vi "Stop Condition - Saturation B-Value (SubVI).vi"(6 "Enum":enum16{"Saturation", "B-Check"}(ring), 8 "error in (no error)":errorcluster, 10 "Time":dbl, 11 "Cluster in":T1 {"M Event" items=["Stop", "Running", "PID", "Up Limit", "Down Limit", "Load Limit"]; "Test Type" items=["Please Select"=0, "Triaxial Shear"=1, "Triaxial UU"=2, "Shearbox"=3, "Permeability"=4, "Consolidation (Stepped Loading)/Swelling"=5, "UCT"=8, "Isotropic Consolidation"=9, "Swelling Pressure"=10, "B-Check"=11, "Saturation (Step Increment)"=12, "Saturation (Ramp)"=13]; "Data"."Test Type" items=["Please Select"=0, "Triaxial Shear"=1, "Triaxial UU"=2, "Shearbox"=3, "Permeability"=4, "Consolidation (Stepped Loading)/Swelling"=5, "UCT"=8, "Isotropic Consolidation"=9, "Swelling Pressure"=10, "B-Check"=11, "Saturation (Step Increment)"=12, "Saturation (Ramp)"=13]}) -> (0 "error IO":errorcluster, 3 "Cluster in 2":T1 {"M Event" items=["Stop", "Running", "PID", "Up Limit", "Down Limit", "Load Limit"]; "Test Type" items=["Please Select"=0, "Triaxial Shear"=1, "Triaxial UU"=2, "Shearbox"=3, "Permeability"=4, "Consolidation (Stepped Loading)/Swelling"=5, "UCT"=8, "Isotropic Consolidation"=9, "Swelling Pressure"=10, "B-Check"=11, "Saturation (Step Increment)"=12, "Saturation (Ramp)"=13]; "Data"."Test Type" items=["Please Select"=0, "Triaxial Shear"=1, "Triaxial UU"=2, "Shearbox"=3, "Permeability"=4, "Consolidation (Stepped Loading)/Swelling"=5, "UCT"=8, "Isotropic Consolidation"=9, "Swelling Pressure"=10, "B-Check"=11, "Saturation (Step Increment)"=12, "Saturation (Ramp)"=13]}, 4 "Log?":bool)   [LabVIEW 2019]
uses:
  Controls/RunTest - Data Structure.ctl
  Controls/Test Panel - Data Structure.ctl
  Controls/Station - Test Type.ctl
  <vilib>/Utility/miscctls.llb/LVRowAndColumnTypeDef.ctl
  Controls/RunTest - Calculate Data.ctl
  <vilib>/httpClient/ClientHandle.ctl
  Controls/RunTest - Start Condition.ctl
  Controls/RunTest - Stop Condition.ctl
  Controls/UDP - Event.ctl
  Controls/eFGV States.ctl
  <vilib>/httpClient/LabVIEWHTTPClient.lvlib
panel:
  in  "Test Run Time":dbl
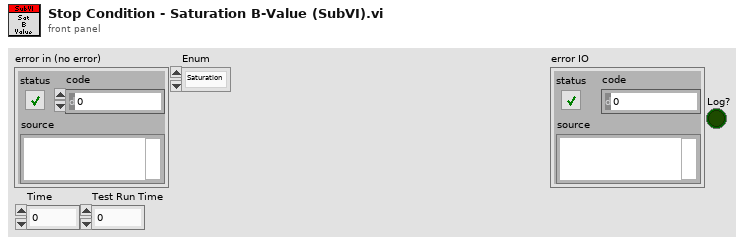
[diagram p1: front panel]
types:
  T1 = typedef "RunTest - Data Structure.ctl" = cluster{"Test Plan":string[], "PlanRow":i32, "Device Name":string[], "Timeout":i32, "Start?":bool, "Pause?":bool, "IP Address":string[], "LogRow":i32, "Logtype":u16, "Log Elapse":sgl, "Data":T2, "Stop log?":bool, "tdms":refnum<k34>, "Sensor Data":sgl[], "Start time":timestamp, "Prev Log Elapse":u32, "Plot":u16, "X-Axis":u16[], "Y-Axis":u16[], "XY":cluster{"X":dbl, "Y":dbl}[][], "End Stage?":bool, "1run":bool, "Condition":u16[], "Start Con":bool, "Log Con":bool, "Stop Con":bool, "Start Elapse":dbl, "Start Load":dbl, "Motor":i32, "StartRow":i32, "number log":i32, "Dir":bool, "Start time test":timestamp, "Auto":bool, "Check return?":bool, "Inv":cluster{"M":i32[], "Bool":bool[]}, "tdms temp":refnum<k34>, "Zero?":bool, "Plot Timer":dbl, "1st Run":bool, "TDMS Path":path, "MaxLoad":dbl, "Log Timer":sgl[], "Test Type":T3, "Log Sensor":string[], "Save?":bool, "1st Log":bool, "Y-Axis 2":u16[], "On Y-Axis 2":bool, "Decimal":u8[], "Init":cluster{"PWP TS":sgl, "Load TS":sgl, "Volume TS":sgl, "Disp TS":sgl, "CP":sgl, "Vol In":sgl, "Vol Out":sgl, "Load UCT":sgl, "Disp UCT":sgl, "PWP Sat":sgl, "CP Sat":sgl, "Volume IsoCons":sgl, "PWP IsoCons":sgl, "PWP TUU":sgl, "Load TUU":sgl, "Volume TUU":sgl, "Disp TUU":sgl, "Load Cons":sgl, "Disp Cons":sgl, "Volume Sat":sgl, "Vertical Load SB":sgl, "Vertical Disp SB":sgl, "H Disp SB":sgl, "H Load SB":sgl, "PWP BC":sgl, "CP BC":sgl, "PWP Sat Step":sgl, "CP Sat Step":sgl, "Volume Sat Step":sgl, "PWP Sat Ramp":sgl, "CP Sat Ramp":sgl, "Volume Sat Ramp":sgl}, "Calc":T5, "Device Index":i32[], "Channel Index":i32[], "http ref":T6, "fileid":string, "Step Cons":cluster{"V Stress":sgl, "H Settlement":sgl}, "RunTest":bool, "Graph Last":i32, "Init?":bool, "Datalog":bool[], "Start":T7, "Stop":T8, "Running?":bool, "StartTime":dbl, "Log Prev Time":dbl, "KeyName":string[], "Test RunTime":dbl, "Log Prev Axial":dbl, "M Event":T9[], "Last Log":bool, "popup":bool, "PreStart UU":bool, "PreStart Sat":bool, "PreStart BC":bool, "PreStart Sat Step":bool, "PreStart Sat Ramp":bool, "Prev Sat IP":string, "IP Device ID":string[]}
  T2 = typedef "Test Panel - Data Structure.ctl" = cluster{"Station":string, "Sample ID":string, "Job No":string, "Job Description":string, "Filename":string, "Test Type":T3, "Speciment No":string, "Depth":string, "Height":string, "Diameter/Length":string, "Weight":string, "Test Parameter":string, "Station[]":string[], "Edit Pos":T4, "Edit Pos Prev":T4, "Area":string, "Path":string, "sample_id":string}
  T3 = typedef "Station - Test Type.ctl" = u16
  T4 = typedef "LVRowAndColumnTypeDef.ctl" = cluster{"Row":i32, "Column":i32}
  T5 = typedef "RunTest - Calculate Data.ctl" = cluster{"TS":cluster{"Change PWP":sgl, "Change Vol":sgl, "Axial Load":sgl, "CiL":sgl, "Deviator":sgl, "Axial Strain":sgl, "MaxDeviator":sgl, "SS":sgl, "CAS":sgl}, "TUU":cluster{"Change PWP":sgl, "Axial Load":sgl, "CiL":sgl, "Deviator":sgl, "Axial Strain":sgl, "MaxDeviator":sgl}, "Sat":cluster{"B Value":sgl, "PWP Diss":sgl, "CPP":sgl, "CV":sgl}, "Per":cluster{"Change Vol In":sgl, "Change Vol Out":sgl, "Mean Vol":sgl, "Gradient Pressure":sgl, "Outlet Flow":sgl, "Inlet Flow":sgl, "I X1":sgl, "I X2":sgl, "I Y1":sgl, "I Y2":sgl, "O X1":sgl, "O X2":sgl, "O Y1":sgl, "O Y2":sgl}, "Step Cons":cluster{"V Stress":sgl, "H Settlement":sgl, "Total H Settle":sgl, "Prev Total H":sgl}, "UCT":cluster{"ALC":sgl, "H Change":sgl, "Deviator":sgl, "Axial Strain":sgl, "V Stress":sgl, "MaxDeviator":sgl}, "ISO Cons":cluster{"CPP":sgl, "PWP Diss":sgl, "CV":sgl, "VS":sgl}, "SB":cluster{"Speci LenC":sgl, "Shear Strain":sgl, "H LC":sgl, "Normal Stress":sgl, "Shear Stress":sgl, "MaxShear":sgl}, "BC":cluster{"B Value":sgl, "PWP Diss":sgl, "CPP":sgl, "CV":sgl}, "Sat Step":cluster{"B Value":sgl, "PWP Diss":sgl, "CPP":sgl, "CV":sgl}, "Sat Ramp":cluster{"B Value":sgl, "PWP Diss":sgl, "CPP":sgl, "CV":sgl}, "Prev Log":string[]}
  T6 = typedef "LabVIEWHTTPClient.lvlib/ClientHandle.ctl" = refnum<k1>
  T7 = typedef "RunTest - Start Condition.ctl" = cluster{"Cons":cluster{"VS":dbl, "Delay":bool, "No Delay":dbl}, "Sat":cluster{"CP":dbl, "BP":dbl, "StartBP":bool, "Target CP":bool, "Target BP":bool}, "Iso":cluster{"Select":dbl, "BP":dbl, "IC2":dbl, "IC3":dbl, "IC4":dbl, ". IC6":bool, "IC6":dbl, "IC6-2":dbl, "Time Cond":dbl, "Last PWP":dbl, "Target CP":bool, "Target BP":bool, "NewCP":dbl, "NewBP":dbl, "Noti CP":bool, "Noti BP":bool, "Noti PWP":bool, "PrevSatBP":dbl}, "TS":cluster{"SS":dbl, "Engage":bool, "ES":dbl, "LC":dbl, "PreStart":bool, "Trig SS":bool, "Drain":dbl, "Select":u16, "Max SS .":bool, "MaxSS":dbl}, "TUU":cluster{"SS":dbl, "Engage":bool, "ES":dbl, "LC":dbl, "PreStart":bool, "Trig SS":bool, "CP":dbl, "Delay Value":dbl, "Delay":bool, "CP PID":bool}, "UCT":cluster{"SS":dbl, "Engage":bool, "ES":dbl, "LC":dbl, "PreStart":bool, "Trig SS":bool}, "Enable?":bool, "SB":cluster{"SS":dbl, "Engage":bool, "ES":dbl, "LC":dbl, "PreStart":bool, "Trig SS":bool, "VS":dbl, "Delay Value":dbl, "Delay":bool, "VS PID":bool}, "Perm":cluster{"DP":dbl}, "BC":cluster{"CP":dbl, "Target CP":bool, "Target BP":bool, "CP Inc":dbl, "CP .Init":bool, "CP Init":dbl, "1st BC":bool}, "Sat (Step)":cluster{"Select":dbl, "CP":dbl, "BP":dbl, "EP":dbl, "StartCP":bool, "Target CP":bool, "Target BP":bool}, "Sat (Ramp)":cluster{"Select":dbl, "CP":dbl, "BP":dbl, "EP":dbl, "StartCP":bool, "Target CP":bool, "Target BP":bool, "Time Rate":u32}}
  T8 = typedef "RunTest - Stop Condition.ctl" = cluster{"Cons":cluster{"Select":i32, "Disp":dbl, "Time":dbl, "Time2":dbl, "Disp 2":dbl, "Time Cond":dbl, "Last Disp":dbl, "Swell":bool, "T50,90,100":cluster{"t50_x_min":dbl, "t50_y_value":dbl, "t90_x_min":dbl, "t90_y_value":dbl, "t100_x_min":dbl, "t100_y_value":dbl, "target_column":string, "test_type":string, "error":string}}, "Sat":cluster{"Select":i32, "PP":dbl, "Time":dbl, "VC":dbl, "Time2":dbl, "Time Cond":dbl, "Last PP":dbl, ".B":bool, "B":dbl, "Last Vc":dbl, "Time Cond 2":dbl, "Time3":dbl, "Time Cond 3":dbl, "B Achieve":bool, "PP Achieve":bool, "VC Achieve":bool, "Max Achieve":bool, "CP Check":dbl, "Skip Next":bool, "B Achieve Stage":u32, ".CP Check":bool}, "Iso":cluster{"PP":dbl, "Time":dbl, "VC":dbl, "Time2":dbl, "Time Cond":dbl, "Last Vc":dbl, ".PP":bool, "Time Cond 2":dbl, "Select":i32, "BS":cluster{"t50_x_min":dbl, "t50_y_value":dbl, "t90_x_min":dbl, "t90_y_value":dbl, "t100_x_min":dbl, "t100_y_value":dbl, "target_column":string, "test_type":string, "error":string}, "Final VC":dbl, "ASTM":cluster{"t50_x_min":dbl, "t50_y_value":dbl, "t90_x_min":dbl, "t90_y_value":dbl, "t100_x_min":dbl, "t100_y_value":dbl, "target_column":string, "test_type":string, "error":string}, "ASTM Log":cluster{"t50_x_min":dbl, "t50_y_value":dbl, "t90_x_min":dbl, "t90_y_value":dbl, "t100_x_min":dbl, "t100_y_value":dbl, "target_column":string, "test_type":string, "error":string}, "PP Achieve":bool, "VC Achieve":bool}, "TS":cluster{"Axial":dbl, ".MaxDev":bool, "MaxDev Value":dbl, "Return":bool, "Reset":bool, "Prev Time":dbl, "PostStop Run":bool, "CP Stop":bool, "BP Stop":bool, "PostStop Trig":bool, "Reset Value":dbl, "BPTrig":bool, "CPTrig":bool, "VLCTrig":bool, "CAxial":dbl, "Select":i32}, "TUU":cluster{"Axial":dbl, ".MaxDev":bool, "MaxDev Value":dbl, "Return":bool, "Reset":bool, "Prev Time":dbl, "PostStop Run":bool, "CP Stop":bool, "BP Stop":bool, "PostStop Trig":bool, "Reset Value":dbl, "BPTrig":bool, "CPTrig":bool, "VLCTrig":bool}, "UCT":cluster{"Axial":dbl, ".MaxDev":bool, "MaxDev Value":dbl, "Return":bool, "Reset":bool, "Prev Time":dbl, "PostStop Run":bool, "CP Stop":bool, "BP Stop":bool, "PostStop Trig":bool}, "Enable?":bool, "SB":cluster{"Shear":dbl, ".MaxShear":bool, "MaxShear Value":dbl, "Return":bool, "Reset":bool, "Prev Time":dbl, "PostStop Run":bool, "CP Stop":bool, "BP Stop":bool, "PostStop Trig":bool, "Reset Value":dbl, "BPTrig":bool, "CPTrig":bool, "VLCTrig":bool}, "Perm":cluster{"Max Time":bool, "Reset":bool, "PostStop Run":bool, "Ratio":bool, "Reset Value":dbl, "Time":dbl, "RatioTime":dbl, "RatioMore":dbl, "RatioLess":dbl, "Time Cond":dbl, "Time Cond 2":dbl, "Prev IF":dbl, "Prev OF":dbl, "PostStop Trig":bool, "BP Trig":bool, "DP Stop":bool, "BP Stop":bool, "CP Stop":bool, "CP Trig":bool}, "SP":cluster{".Max Time":bool, ".Time":bool, "Time":dbl, "MaxTime":dbl, "Time Cond":dbl, "Max Time Cond":dbl, "Stress":dbl}, "BC":cluster{"Select":i32, "PP":dbl, "Time":dbl, "Time Cond":dbl, "Last PP":dbl, ".B":bool, "B":dbl, "Time 2":dbl, "Time Cond 2":dbl, "B Achieve":bool, "PP Achieve":bool, "Max Achieve":bool, "CP Check":dbl, "Skip Next":bool, "B Achieve Stage":u32, ".CP Check":bool}, "Sat (Step)":cluster{"Select":i32, "PP":dbl, "Time":dbl, "VC":dbl, "Time2":dbl, "Time Cond":dbl, "Last PP":dbl, ".B":bool, "B":dbl, "Last Vc":dbl, "Time Cond 2":dbl, "Time3":dbl, "Time Cond 3":dbl, "B Achieve":bool, "PP Achieve":bool, "VC Achieve":bool, "Max Achieve":bool, "CP Check":dbl, "Skip Next":bool, "B Achieve Stage":u32}, "Sat (Ramp)":cluster{"Select":i32, "PP":dbl, "Time":dbl, "VC":dbl, "Time2":dbl, "Time Cond":dbl, "Last PP":dbl, ".B":bool, "B":dbl, "Last Vc":dbl, "Time Cond 2":dbl, "Time3":dbl, "Time Cond 3":dbl, "B Achieve":bool, "PP Achieve":bool, "VC Achieve":bool, "Max Achieve":bool, "CP Check":dbl, "Skip Next":bool, "B Achieve Stage":u32}}
  T9 = typedef "UDP - Event.ctl" = u16
  T10 = typedef "eFGV States.ctl" = enum16{"Init", "Read", "Write", "Exit"}
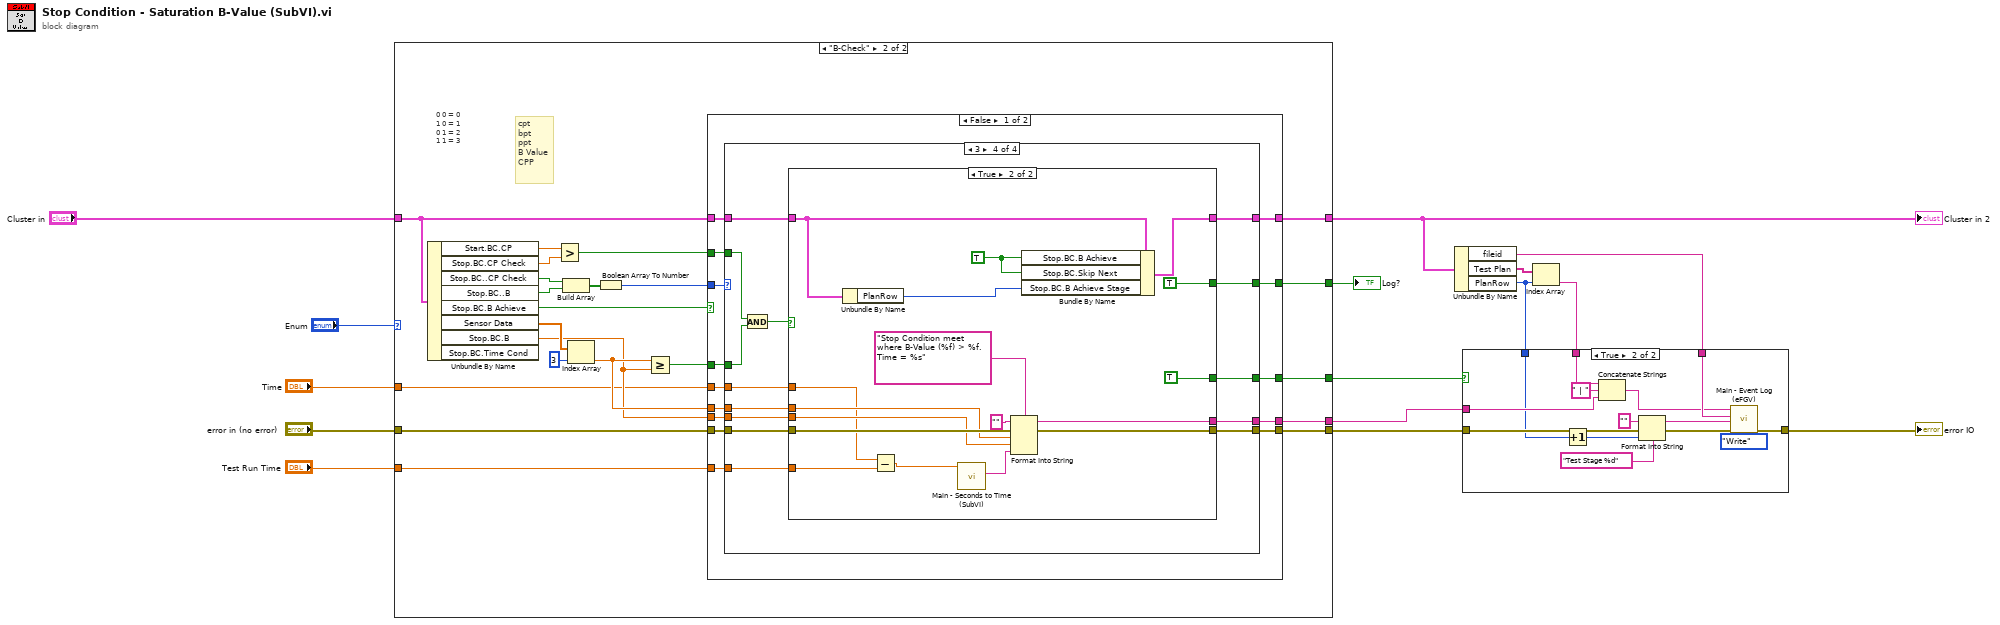
[diagram p0: block diagram]
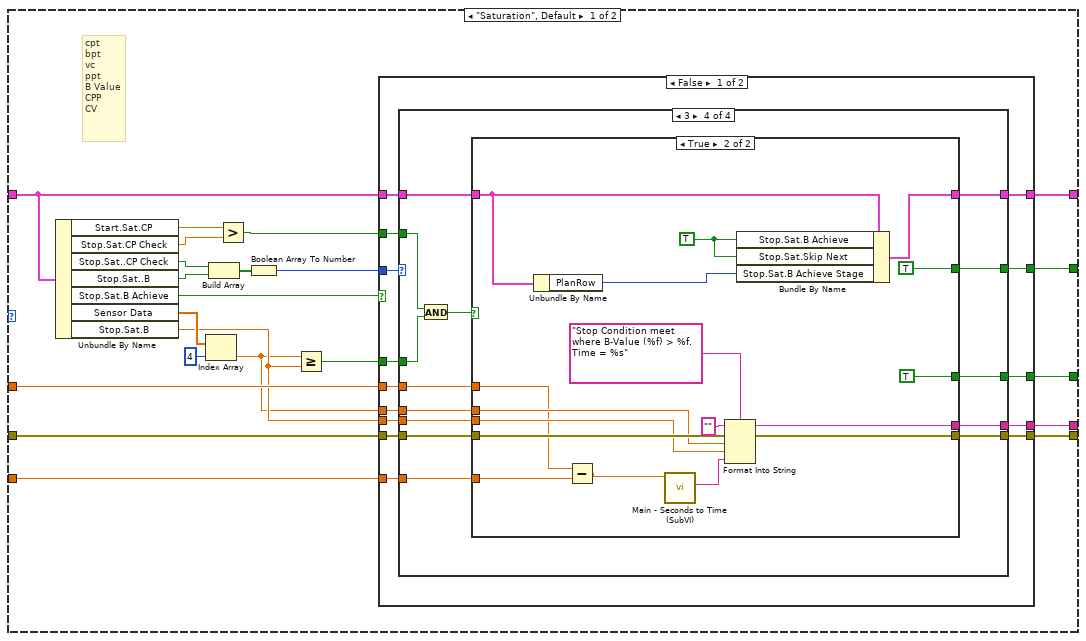
[diagram p2: hidden frame]
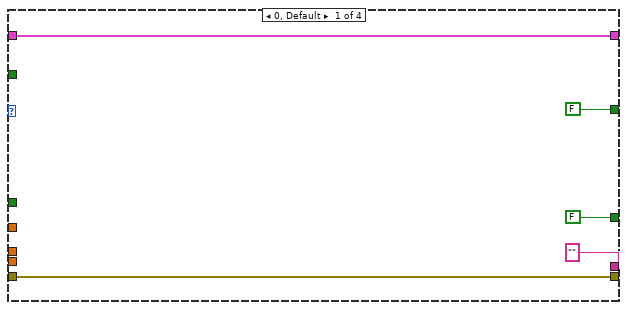
[diagram p3: hidden frame]
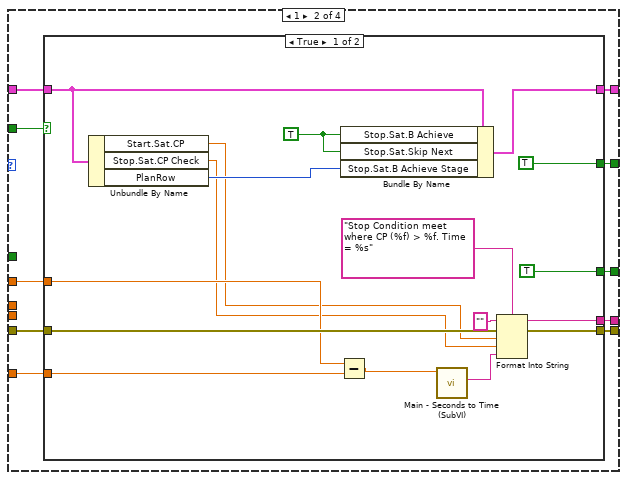
[diagram p4: hidden frame]
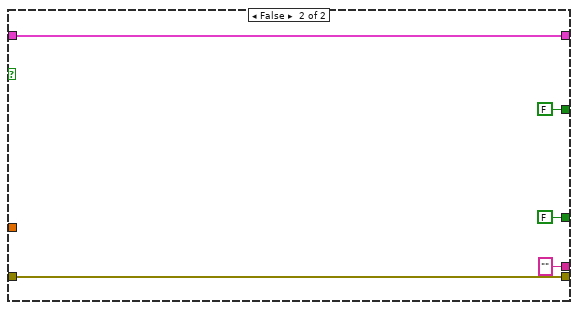
[diagram p5: hidden frame]
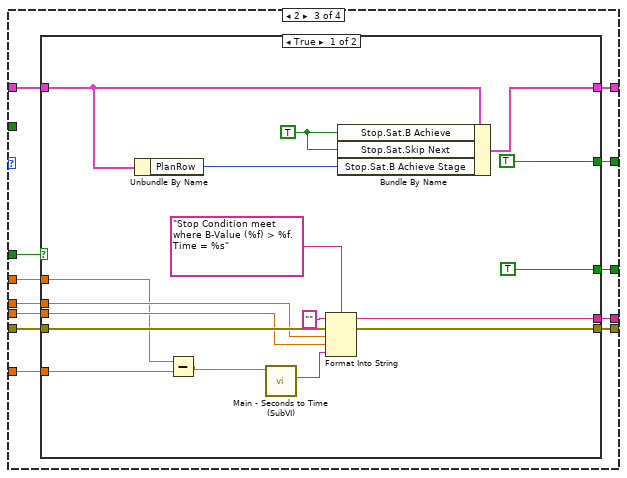
[diagram p6: hidden frame]
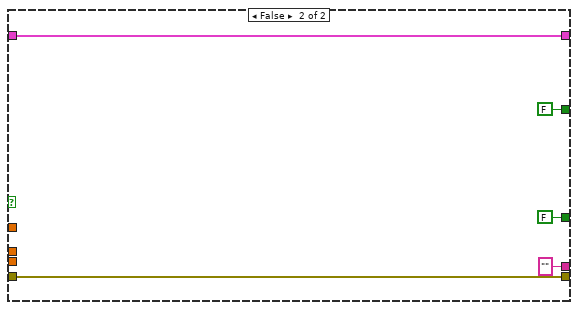
[diagram p7: hidden frame]
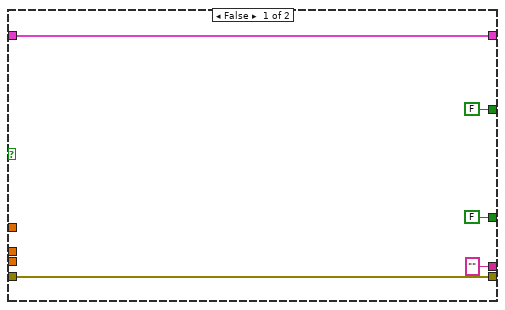
[diagram p8: hidden frame]
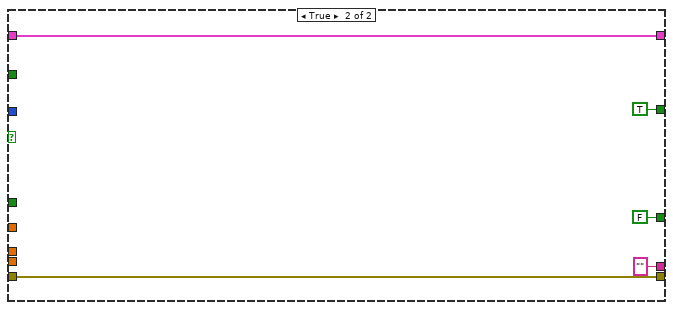
[diagram p9: hidden frame]
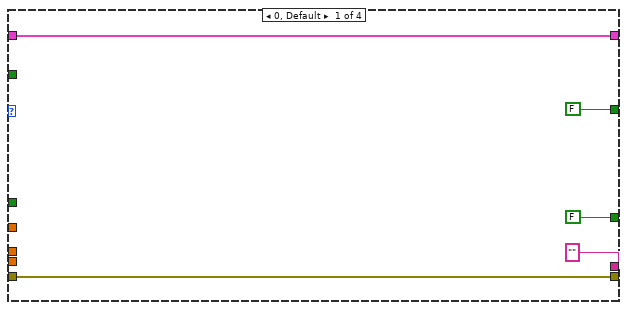
[diagram p10: hidden frame]
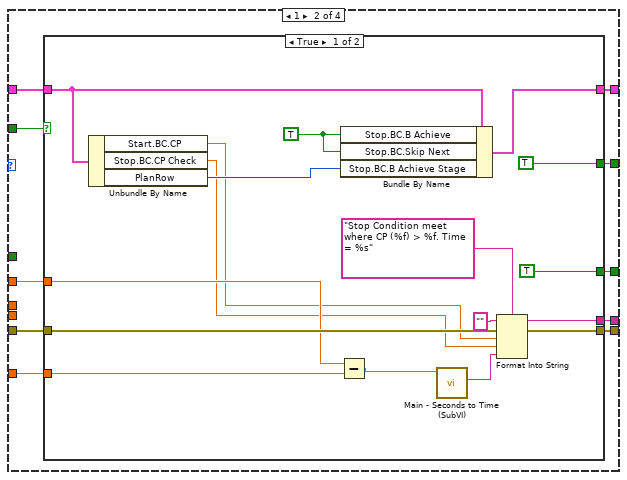
[diagram p11: hidden frame]
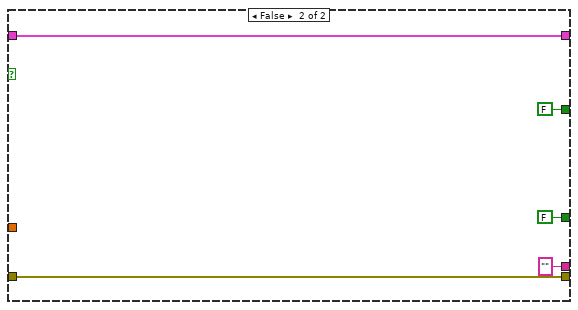
[diagram p12: hidden frame]
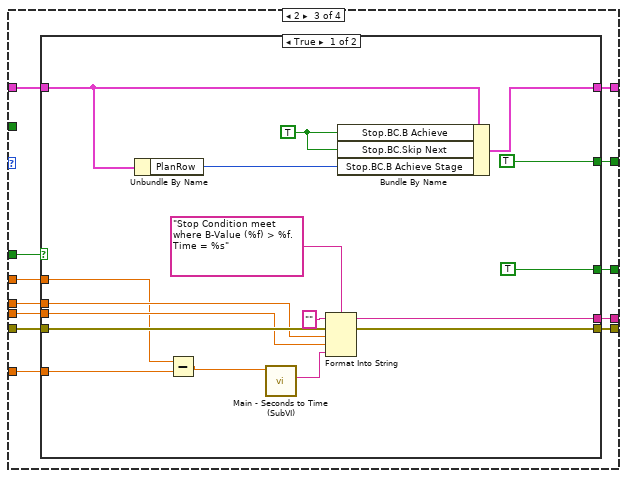
[diagram p13: hidden frame]
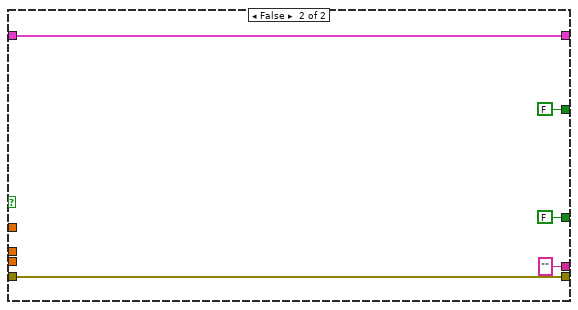
[diagram p14: hidden frame]
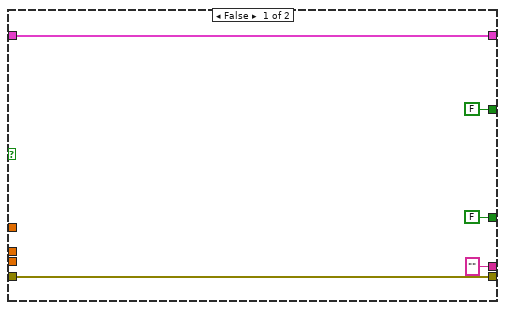
[diagram p15: hidden frame]
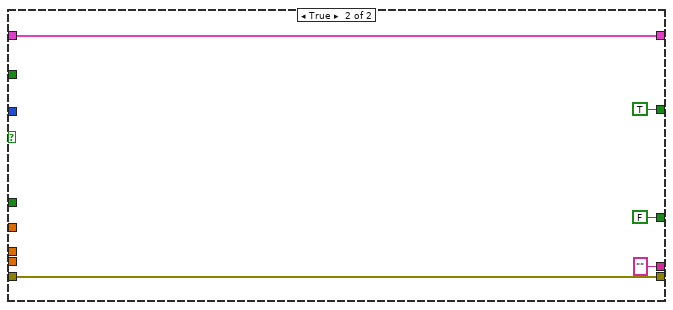
[diagram p16: hidden frame]
diagram:
  n1 = case shown="\"B-Check\"" "Enum" {
    tunnel: "Cluster in" -> [w30 w176]
    tunnel: "error in (no error)" -> [w35 w172]
    tunnel: "Time" -> [w33 w164]
    tunnel: [w21 w175] -> w12
    tunnel: [w18 w173] -> w7
    tunnel: [w20 w174] -> w6
    tunnel: [w22 w177] -> w5
    tunnel: [w19 w171] -> w3
    tunnel: "Test Run Time" -> [w34 w169]
    frame "Saturation", Default {
      # "cpt\nbpt\nvc\nppt\nB Value\nCPP\nCV"
      n2 = Unbundle By Name(w30) -> ("Start.Sat.CP"=w32:dbl, "Stop.Sat.CP Check"=w31:dbl, "Stop.Sat..CP Check"=w25:bool, "Stop.Sat..B"=w24:bool, "Stop.Sat.B Achieve"=w27:bool, "Sensor Data"=w37:sgl[], "Stop.Sat.B"=w17:dbl)
      n3 = Index Array(array=w37, index=4) -> (element=w16:sgl)
      n4 = Build Array(w25, w24) -> (w26:bool[])
      n5 = Greater?(x=w32, y=w31) -> (0:w29:bool)
      n6 = Boolean Array To Number(Boolean array=w26) -> (number=w23:u32)
      n7 = Greater Or Equal?(x=w16, y=w17) -> (x >= y?=w28:bool)
      n8 = case shown="False" w27 {
        tunnel: w23 -> [w51 _]
        tunnel: [w50 w163] -> w22
        tunnel: w30 -> [w49 w163]
        tunnel: [w48 TRUE] -> w21
        tunnel: [w47 FALSE] -> w20
        tunnel: [w46 w160] -> w18
        tunnel: w35 -> [w45 w160]
        tunnel: [w44 ""] -> w19
        tunnel: w29 -> [w43 _]
        tunnel: w33 -> [w42 _]
        tunnel: w34 -> [w41 _]
        tunnel: w28 -> [w40 _]
        tunnel: w16 -> [w39 _]
        tunnel: w17 -> [w38 _]
        frame False {
          n9 = case shown="3" w51 {
            tunnel: [w56 w65 w99 w129] -> w50
            tunnel: w49 -> [w56 w66 w100 w130]
            tunnel: [FALSE w64 w97 w128] -> w48
            tunnel: [FALSE w63 w96 w127] -> w47
            tunnel: [w53 w61 w94 w135] -> w46
            tunnel: w45 -> [w53 w60 w93 w136]
            tunnel: ["" w62 w95 w126] -> w44
            tunnel: w43 -> [_ w59 _ w125]
            tunnel: w42 -> [_ w58 w92 w131]
            tunnel: w41 -> [_ w57 w91 w132]
            tunnel: w40 -> [_ _ w98 w124]
            tunnel: w39 -> [_ _ w90 w134]
            tunnel: w38 -> [_ _ w89 w133]
            frame 0, Default {
            }
            frame 1 {
              n10 = case shown="True" w59 {
                tunnel: [w81 w85] -> w61
                tunnel: w60 -> [w82 w85]
                tunnel: [w83 w88] -> w65
                tunnel: w66 -> [w77 w88]
                tunnel: [w79 ""] -> w62
                tunnel: [TRUE FALSE] -> w63
                tunnel: w58 -> [w76 _]
                tunnel: [TRUE FALSE] -> w64
                tunnel: w57 -> [w75 _]
                frame True {
                  w67 = TRUE ("Stop.Sat.B Achieve")
                  n11 = Unbundle By Name(w77) -> ("Start.Sat.CP"=w73:dbl, "Stop.Sat.CP Check"=w72:dbl, "PlanRow"=w74:i32)
                  n12 = Subtract(x=w76, y=w75) -> (x-y=w68:dbl)
                  n13 = Bundle By Name(cluster=w77, "Stop.Sat.B Achieve"=w67, "Stop.Sat.Skip Next"=w67, "Stop.Sat.B Achieve Stage"=w74) -> (w83:T1)
                  n14 = call "Main - Seconds to Time (SubVI).vi"("Seconds"=w68) -> ("Time string"=w69:string)  [unwired: 9 in, 1 out]
                  n15 = Format Into String(format string="Stop Condition meet where CP (%f) > %f. Time = %s", initial string="", error in=w82, w73, w72, w69) -> (resulting string=w79:string, error out=w81:errorcluster)
                }
                frame False {
                }
              }
            }
            frame 2 {
              n16 = case shown="True" w98 {
                tunnel: [w115 w121] -> w94
                tunnel: w93 -> [w116 w121]
                tunnel: [w117 w122] -> w99
                tunnel: w100 -> [w109 w122]
                tunnel: w89 -> [w114 _]
                tunnel: w90 -> [w113 _]
                tunnel: [w111 ""] -> w95
                tunnel: [TRUE FALSE] -> w96
                tunnel: w92 -> [w108 _]
                tunnel: [TRUE FALSE] -> w97
                tunnel: w91 -> [w107 _]
                frame True {
                  w101 = TRUE ("Stop.Sat.B Achieve")
                  n17 = Unbundle By Name(w109) -> ("PlanRow"=w103:i32)
                  n18 = Subtract(x=w108, y=w107) -> (x-y=w102:dbl)
                  n19 = call "Main - Seconds to Time (SubVI).vi"("Seconds"=w102) -> ("Time string"=w104:string)  [unwired: 9 in, 1 out]
                  n20 = Format Into String(format string="Stop Condition meet where B-Value (%f) > %f. Time = %s", initial string="", error in=w116, w113, w114, w104) -> (resulting string=w111:string, error out=w115:errorcluster)
                  n21 = Bundle By Name(cluster=w109, "Stop.Sat.B Achieve"=w101, "Stop.Sat.Skip Next"=w101, "Stop.Sat.B Achieve Stage"=w103) -> (w117:T1)
                }
                frame False {
                }
              }
            }
            frame 3 {
              n22 = And(x=w125, y=w124) -> (x .and. y?=w123:bool)
              n23 = case shown="True" w123 {
                tunnel: [w141 w158] -> w129
                tunnel: w136 -> [w138 w155]
                tunnel: [w138 w154] -> w135
                tunnel: w133 -> [_ w153]
                tunnel: w134 -> [_ w152]
                tunnel: [FALSE TRUE] -> w127
                tunnel: ["" w149] -> w126
                tunnel: [FALSE TRUE] -> w128
                tunnel: w130 -> [w141 w147]
                tunnel: w131 -> [_ w144]
                tunnel: w132 -> [_ w143]
                frame False {
                }
                frame True {
                  w142 = TRUE ("Stop.Sat.B Achieve")
                  n24 = Unbundle By Name(w147) -> ("PlanRow"=w146:i32)
                  n25 = Subtract(x=w144, y=w143) -> (x-y=w145:dbl)
                  n26 = call "Main - Seconds to Time (SubVI).vi"("Seconds"=w145) -> ("Time string"=w150:string)  [unwired: 9 in, 1 out]
                  n27 = Format Into String(format string="Stop Condition meet where B-Value (%f) > %f. Time = %s", initial string="", error in=w155, w152, w153, w150) -> (resulting string=w149:string, error out=w154:errorcluster)
                  n28 = Bundle By Name(cluster=w147, "Stop.Sat.B Achieve"=w142, "Stop.Sat.Skip Next"=w142, "Stop.Sat.B Achieve Stage"=w146) -> (w158:T1)
                }
              }
            }
          }
        }
        frame True {
        }
      }
    }
    frame "B-Check" {
      # "0 0 = 0\n1 0 = 1\n0 1 = 2\n1 1 = 3"
      # "cpt\nbpt\nppt\nB Value\nCPP"
      n29 = Unbundle By Name(w176) -> ("Start.BC.CP"=w183:dbl, "Stop.BC.CP Check"=w182:dbl, "Stop.BC..CP Check"=w181:bool, "Stop.BC..B"=w180:bool, "Stop.BC.B Achieve"=w165:bool, "Sensor Data"=w185:sgl[], "Stop.BC.B"=w166:dbl)  [unwired: 1 out]
      n30 = Greater?(x=w183, y=w182) -> (0:w170:bool)
      n31 = Build Array(w181, w180) -> (w179:bool[])
      n32 = Index Array(array=w185, index=3) -> (element=w167:sgl)
      n33 = Boolean Array To Number(Boolean array=w179) -> (number=w178:u32)
      n34 = Greater Or Equal?(x=w167, y=w166) -> (x >= y?=w168:bool)
      n35 = case shown="False" w165 {
        tunnel: w178 -> [w199 _]
        tunnel: [w198 w311] -> w177
        tunnel: w176 -> [w197 w311]
        tunnel: [w196 TRUE] -> w175
        tunnel: [w195 FALSE] -> w174
        tunnel: [w194 w308] -> w173
        tunnel: w172 -> [w193 w308]
        tunnel: [w192 ""] -> w171
        tunnel: w170 -> [w191 _]
        tunnel: w164 -> [w190 _]
        tunnel: w169 -> [w189 _]
        tunnel: w168 -> [w188 _]
        tunnel: w167 -> [w187 _]
        tunnel: w166 -> [w186 _]
        frame False {
          n36 = case shown="3" w199 {
            tunnel: [w204 w213 w247 w277] -> w198
            tunnel: w197 -> [w204 w214 w248 w278]
            tunnel: [FALSE w212 w245 w276] -> w196
            tunnel: [FALSE w211 w244 w275] -> w195
            tunnel: [w201 w209 w242 w283] -> w194
            tunnel: w193 -> [w201 w208 w241 w284]
            tunnel: ["" w210 w243 w274] -> w192
            tunnel: w191 -> [_ w207 _ w273]
            tunnel: w190 -> [_ w206 w240 w279]
            tunnel: w189 -> [_ w205 w239 w280]
            tunnel: w188 -> [_ _ w246 w272]
            tunnel: w187 -> [_ _ w238 w282]
            tunnel: w186 -> [_ _ w237 w281]
            frame 0, Default {
            }
            frame 1 {
              n37 = case shown="True" w207 {
                tunnel: [w229 w233] -> w209
                tunnel: w208 -> [w230 w233]
                tunnel: [w231 w236] -> w213
                tunnel: w214 -> [w225 w236]
                tunnel: [w227 ""] -> w210
                tunnel: [TRUE FALSE] -> w211
                tunnel: w206 -> [w224 _]
                tunnel: [TRUE FALSE] -> w212
                tunnel: w205 -> [w223 _]
                frame True {
                  w215 = TRUE ("Stop.Sat.B Achieve")
                  n38 = Unbundle By Name(w225) -> ("Start.BC.CP"=w221:dbl, "Stop.BC.CP Check"=w220:dbl, "PlanRow"=w222:i32)
                  n39 = Subtract(x=w224, y=w223) -> (x-y=w216:dbl)
                  n40 = Bundle By Name(cluster=w225, "Stop.BC.B Achieve"=w215, "Stop.BC.Skip Next"=w215, "Stop.BC.B Achieve Stage"=w222) -> (w231:T1)
                  n41 = call "Main - Seconds to Time (SubVI).vi"("Seconds"=w216) -> ("Time string"=w217:string)  [unwired: 9 in, 1 out]
                  n42 = Format Into String(format string="Stop Condition meet where CP (%f) > %f. Time = %s", initial string="", error in=w230, w221, w220, w217) -> (resulting string=w227:string, error out=w229:errorcluster)
                }
                frame False {
                }
              }
            }
            frame 2 {
              n43 = case shown="True" w246 {
                tunnel: [w263 w269] -> w242
                tunnel: w241 -> [w264 w269]
                tunnel: [w265 w270] -> w247
                tunnel: w248 -> [w257 w270]
                tunnel: w237 -> [w262 _]
                tunnel: w238 -> [w261 _]
                tunnel: [w259 ""] -> w243
                tunnel: [TRUE FALSE] -> w244
                tunnel: w240 -> [w256 _]
                tunnel: [TRUE FALSE] -> w245
                tunnel: w239 -> [w255 _]
                frame True {
                  w249 = TRUE ("Stop.Sat.B Achieve")
                  n44 = Unbundle By Name(w257) -> ("PlanRow"=w251:i32)
                  n45 = Subtract(x=w256, y=w255) -> (x-y=w250:dbl)
                  n46 = call "Main - Seconds to Time (SubVI).vi"("Seconds"=w250) -> ("Time string"=w252:string)  [unwired: 9 in, 1 out]
                  n47 = Format Into String(format string="Stop Condition meet where B-Value (%f) > %f. Time = %s", initial string="", error in=w264, w261, w262, w252) -> (resulting string=w259:string, error out=w263:errorcluster)
                  n48 = Bundle By Name(cluster=w257, "Stop.BC.B Achieve"=w249, "Stop.BC.Skip Next"=w249, "Stop.BC.B Achieve Stage"=w251) -> (w265:T1)
                }
                frame False {
                }
              }
            }
            frame 3 {
              n49 = And(x=w273, y=w272) -> (x .and. y?=w271:bool)
              n50 = case shown="True" w271 {
                tunnel: [w289 w306] -> w277
                tunnel: w284 -> [w286 w303]
                tunnel: [w286 w302] -> w283
                tunnel: w281 -> [_ w301]
                tunnel: w282 -> [_ w300]
                tunnel: [FALSE TRUE] -> w275
                tunnel: ["" w297] -> w274
                tunnel: [FALSE TRUE] -> w276
                tunnel: w278 -> [w289 w295]
                tunnel: w279 -> [_ w292]
                tunnel: w280 -> [_ w291]
                frame False {
                }
                frame True {
                  w290 = TRUE ("Stop.Sat.B Achieve")
                  n51 = Unbundle By Name(w295) -> ("PlanRow"=w294:i32)
                  n52 = Subtract(x=w292, y=w291) -> (x-y=w293:dbl)
                  n53 = call "Main - Seconds to Time (SubVI).vi"("Seconds"=w293) -> ("Time string"=w298:string)  [unwired: 9 in, 1 out]
                  n54 = Format Into String(format string="Stop Condition meet where B-Value (%f) > %f. Time = %s", initial string="", error in=w303, w300, w301, w298) -> (resulting string=w297:string, error out=w302:errorcluster)
                  n55 = Bundle By Name(cluster=w295, "Stop.BC.B Achieve"=w290, "Stop.BC.Skip Next"=w290, "Stop.BC.B Achieve Stage"=w294) -> (w306:T1)
                }
              }
            }
          }
        }
        frame True {
        }
      }
    }
  }
  "Cluster in 2" <- w5
  "Log?" <- w12
  n56 = Unbundle By Name(w5) -> ("fileid"=w9:string, "Test Plan"=w10:string[], "PlanRow"=w8:i32)
  n57 = Index Array(array=w10, index=w8) -> (element=w11:string)
  n58 = case shown="True" w6 {
    tunnel: w7 -> [w312 w316]
    tunnel: [w312 w325] -> w4
    tunnel: w9 -> [_ w324]
    tunnel: w3 -> [_ w320]
    tunnel: w11 -> [_ w323]
    tunnel: w8 -> [_ w314]
    frame False {
    }
    frame True {
      n59 = Increment(x=w314) -> (x+1=w318:i32)
      n60 = Concatenate Strings(w323, " | " ("string"), w320) -> (w321:string)
      n61 = Format Into String(format string="Test Stage %d", initial string="", error in=w316, w318) -> (resulting string=w315:string, error out=w317:errorcluster)
      n62 = call "Main - Event Log (eFGV).vi"("Action"=eFGV_States."Write", "error in"=w317, "Stage"=w315, "Fileid"=w324, "Data In"=w321) -> ("error out"=w325:errorcluster)  [unwired: 3 in, 3 out]
    }
  }
  "error IO" <- w4
